vi "Enregis fichier local.vi"() -> ()   [LabVIEW 2022 SP3]
uses:
  Fichier local.ctl
  Enum/Enum f2l.ctl
  Fichier distant.ctl
  Variables globales/Variable glob generale.vi
panel:
  out "Fichier local":T1
  out "Ensemble données":string[](array[string])
  out "chemin local":path
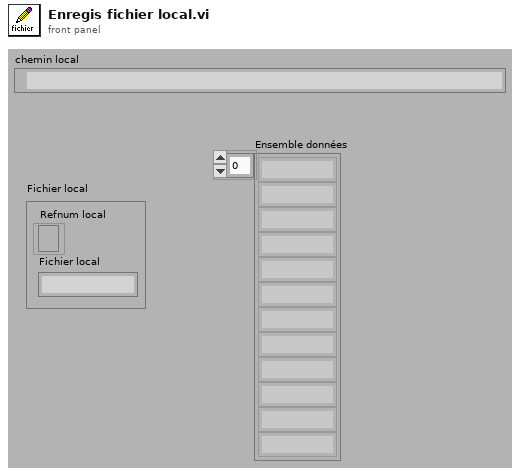
[diagram p1: front panel]
types:
  T1 = typedef "Fichier local.ctl" = cluster{"Refnum local":refnum<file>, "Fichier local":string}
  T2 = typedef "Enum f2l.ctl" = enum16{"Créer dossier local", "Créer fichier local", "Test date", "Test temps", "Données complètes", "Enregistrement"}
  T3 = enum16{"open", "replace", "create", "open or create", "replace or create", "replace or create with confirmation"}
  T4 = typedef "Fichier distant.ctl" = cluster{"refnum distant":refnum<file>, "Fichier distant":string}
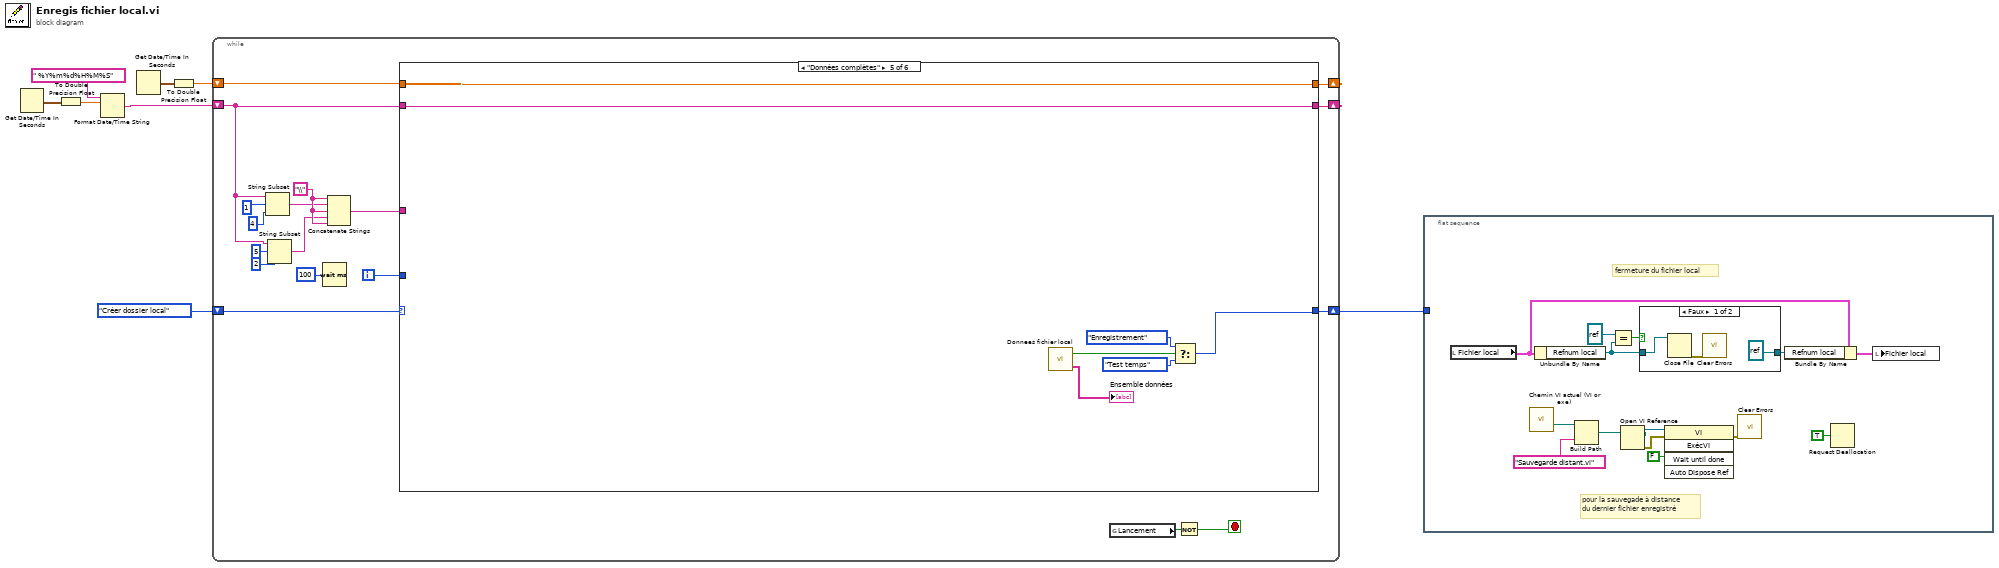
[diagram p0: block diagram]
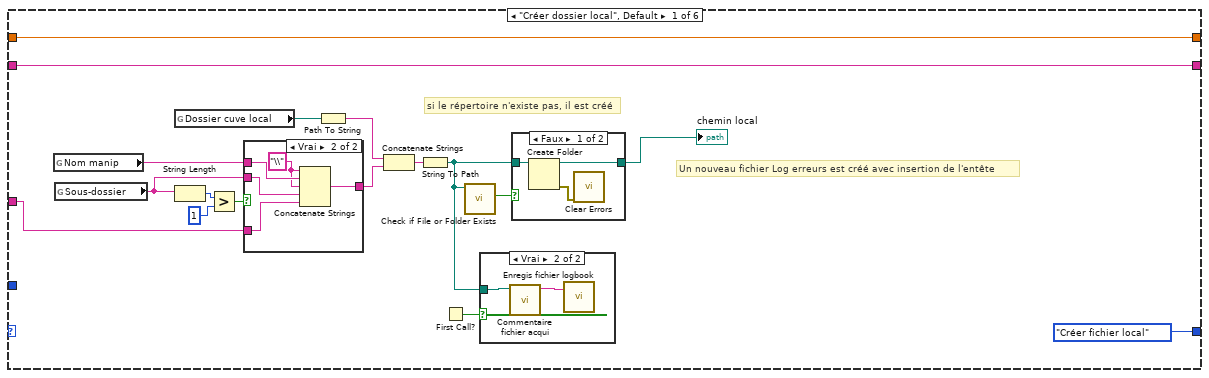
[diagram p3: hidden frame]
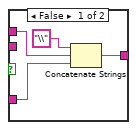
[diagram p5: hidden frame]
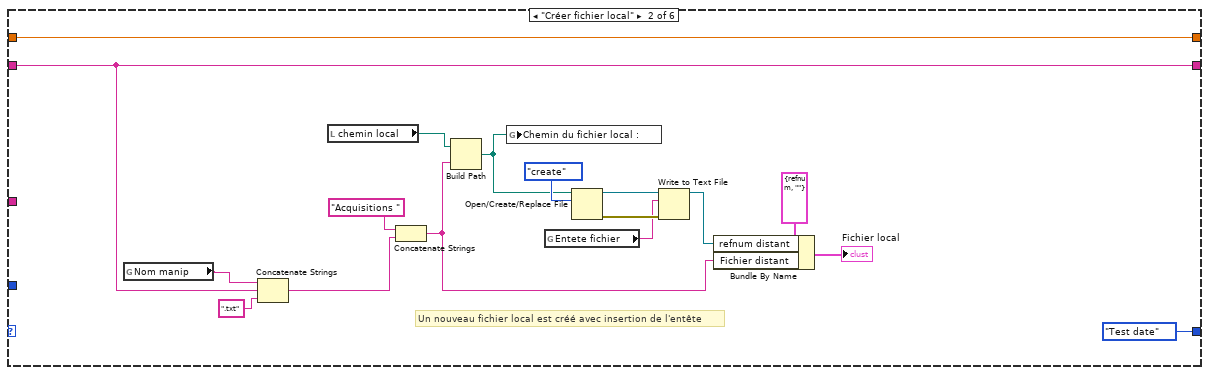
[diagram p7: hidden frame]
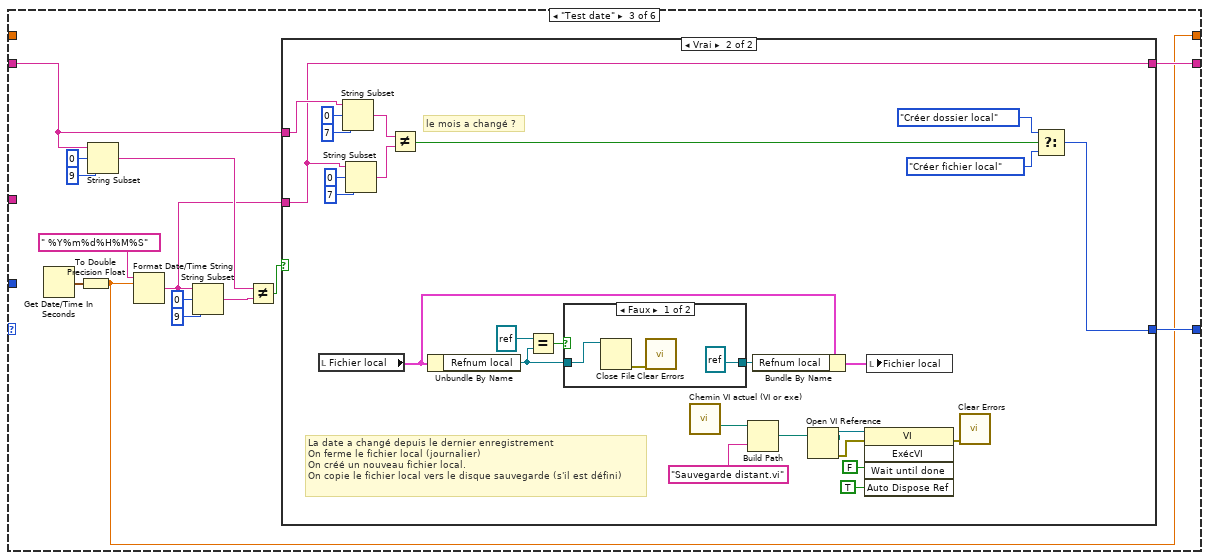
[diagram p8: hidden frame]
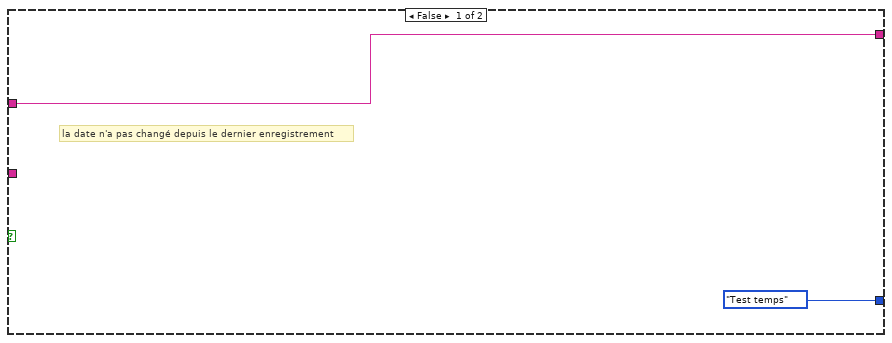
[diagram p9: hidden frame]
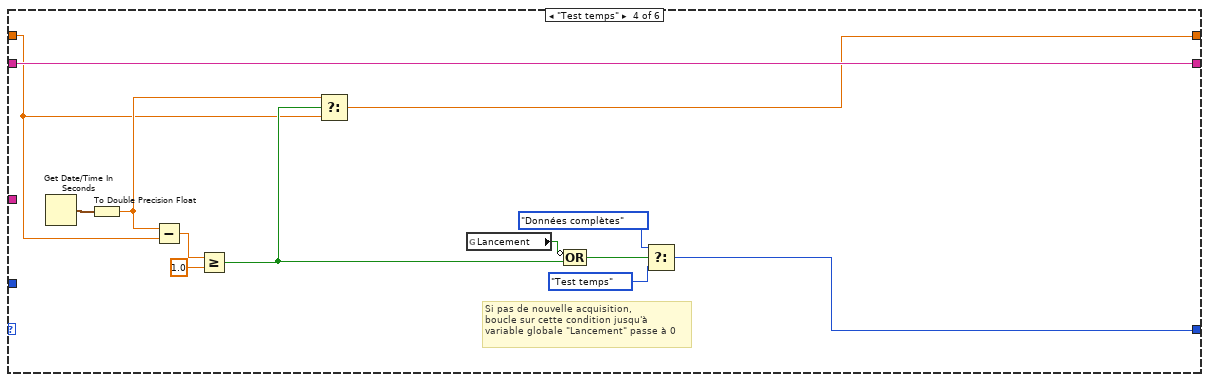
[diagram p11: hidden frame]
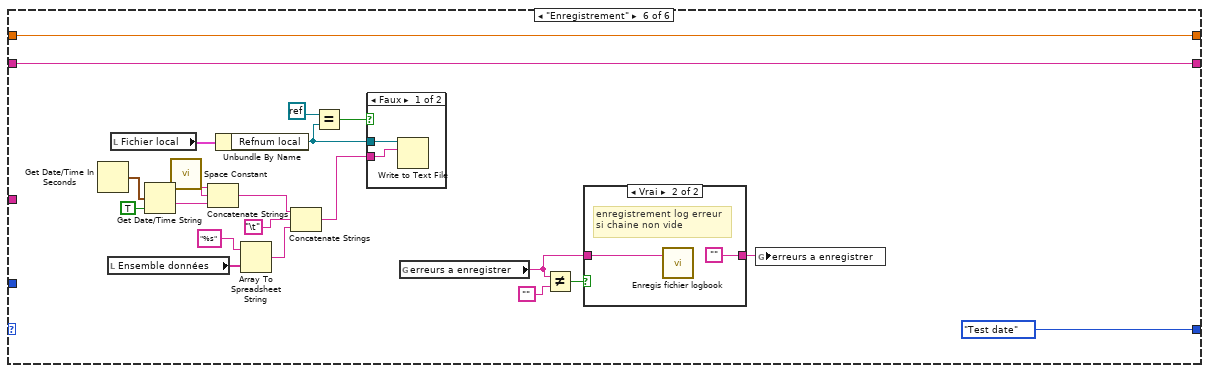
[diagram p12: hidden frame]
diagram:
  n1 = Get Date/Time In Seconds() -> (seconds since 1Jan1904=w7:timestamp)
  n2 = To Double Precision Float(number=w7) -> (double precision float=w5:dbl)
  n3 = Format Date/Time String(time format string (%c)=" %Y%m%d%H%M%S" ("chaîne de format de l'heure (%c)"), seconds (now)=w5) -> (date/time string=w4:string)  [unwired: 1 in]
  n4 = Get Date/Time In Seconds() -> (seconds since 1Jan1904=w3:timestamp)
  n5 = To Double Precision Float(number=w3) -> (double precision float=w2:dbl)
  n6 = while {
    shift-right: [w23] -> _
    shift-left: w4 -> [w13]
    shift-right: [w21] -> _
    shift-left: w2 -> [w22]
    shift-right: [w25] -> w1
    shift-left: Enum_f2l."Créer dossier local" ("Énum") -> [w26]
    i -> [w11]
    stop <- w9 stop-if-true
    w20 = "\\" ("chaîne")
    n7 = String Subset(string=w13, offset (0)=1, length (rest)=4 ("longueur (reste)")) -> (substring=w15:string)
    n8 = String Subset(string=w13, offset (0)=5, length (rest)=2 ("longueur (reste)")) -> (substring=w17:string)
    n9 = Wait (ms)(milliseconds to wait=u32 100 ("attente (ms)")) -> ()  [unwired: 1 out]
    n10 = Concatenate Strings(w20, w15, w20, w17, w20) -> (w12:string)
    n11 = case shown="\"Données complètes\"" w26 {
      tunnel: w12 -> [w34 _ _ _ _ _]
      tunnel: w13 -> [w31 w71 w83 w129 w139 w162]
      tunnel: [Enum_f2l."Créer fichier local" ("Énum") Enum_f2l."Test date" ("Énum") w86 w132 w141 Enum_f2l."Test date" ("Énum")] -> w25
      tunnel: [w31 w71 w85 w129 w139 w162] -> w23
      tunnel: w22 -> [w33 w74 _ w124 w140 w156]
      tunnel: [w33 w74 w84 w123 w140 w156] -> w21
      tunnel: w11 -> [_ _ _ _ _ _]
      frame "Créer dossier local", Default {
        # "Un nouveau fichier Log erreurs est créé avec insertion de l'entête"
        # "si le répertoire n'existe pas, il est créé"
        n12 = global read "Variable glob generale.vi" "Nom manip"() -> (w29:string)
        n13 = global read "Variable glob generale.vi" "Sous-dossier"() -> (w30:string)
        n14 = global read "Variable glob generale.vi" "Dossier cuve local"() -> (w39:path)
        n15 = String Length(string=w30) -> (length=w41:i32)
        n16 = Greater?(x=w41, y=1) -> (0:w40:bool)
        n17 = case shown="Vrai" w40 {
          tunnel: w29 -> [w48 w54]
          tunnel: w30 -> [_ w52]
          tunnel: w34 -> [w47 w51]
          tunnel: [w46 w50] -> w37
          frame False {
            n18 = Concatenate Strings("\\", w48, w47) -> (w46:string)
          }
          frame True {
            w53 = "\\"
            n19 = Concatenate Strings(w53, w54, w53, w52, w51) -> (w50:string)
          }
        }
        n20 = Path To String(path=w39) -> (string=w38:string)
        n21 = Concatenate Strings(w38, w37) -> (w36:string)
        n22 = String To Path(string=w36) -> (path=w27:path)
        n23 = First Call?() -> (First Call?: T/F=w28:bool)
        n24 = call <vilib>:"Check if File or Folder Exists.vi"("path"=w27) -> ("file or folder exists?"=w42:bool)  [unwired: 8 in, 2 out]
        n25 = case shown="Vrai" w28 {
          tunnel: w27 -> [_ w45]
          frame False {
          }
          frame True {
            n26 = call "Commentaire fichier acqui.vi"("Chemin"=w45) -> ("Chaîne"=w44:string)  [unwired: 10 in]
            n27 = call "Enregis fichier logbook.vi"("Chaîne"=w44) -> ()  [unwired: 2 in, 1 out]
          }
        }
        n28 = case shown="Faux" w42 {
          tunnel: w27 -> [w57 w58]
          tunnel: [w56 w58] -> w32
          frame False {
            n29 = Create Folder(path (use dialog)=w57) -> (created path=w56:path, error out=w55:errorcluster)  [unwired: 2 in, 1 out]
            n30 = call <vilib>:"Clear Errors.vi"("error in (no error)"=w55) -> ()  [unwired: 5 in, 2 out]
          }
          frame True {
          }
        }
        "chemin local" <- w32
      }
      frame "Créer fichier local" {
        # "Un nouveau fichier local est créé avec insertion de l'entête"
        n31 = global read "Variable glob generale.vi" "Nom manip"() -> (w73:string)
        n32 = Concatenate Strings(w73, w71, ".txt" ("chaîne")) -> (w61:string)
        n33 = local read "chemin local"() -> (w60:path)
        n34 = Concatenate Strings("Acquisitions ", w61) -> (w62:string)
        n35 = Build Path(base path=w60, name or relative path=w62) -> (appended path=w65:path)
        n36 = global write "Variable glob generale.vi" "Chemin du fichier local :"(w65) -> ()
        n37 = global read "Variable glob generale.vi" "Entete fichier"() -> (w59:string)
        n38 = Open/Create/Replace File(file path (use dialog)=w65, operation (0:open)=T3."create" ("opération (0 : open)")) -> (refnum out=w66:refnum<file>, error out=w67:errorcluster)  [unwired: 1 in, 4 out]
        n39 = Write to Text File(file (use dialog)=w66, text=w59, error in=w67) -> (refnum out=w70:refnum<file>)  [unwired: 1 in, 2 out]
        n40 = Bundle By Name(cluster=T4 {"refnum distant"=refnum, "Fichier distant"=""} ("Refnum File"), "refnum distant"=w70, "Fichier distant"=w62) -> (→"Fichier local":T4)
      }
      frame "Test date" {
        n41 = Get Date/Time In Seconds() -> (seconds since 1Jan1904=w88:timestamp)
        n42 = To Double Precision Float(number=w88) -> (double precision float=w84:dbl)
        n43 = String Subset(string=w83, offset (0)=0, length (rest)=9 ("longueur (reste)")) -> (substring=w78:string)
        n44 = Format Date/Time String(time format string (%c)=" %Y%m%d%H%M%S" ("chaîne de format de l'heure (%c)"), seconds (now)=w84) -> (date/time string=w76:string)  [unwired: 1 in]
        n45 = String Subset(string=w76, offset (0)=0, length (rest)=9 ("longueur (reste)")) -> (substring=w77:string)
        n46 = Not Equal?(x=w78, y=w77) -> (x != y?=w87:bool)
        n47 = case shown="Vrai" w87 {
          tunnel: [Enum_f2l."Test temps" ("Énum") w92] -> w86
          tunnel: w83 -> [w90 w99]
          tunnel: [w90 w98] -> w85
          tunnel: w76 -> [_ w98]
          frame False {
            # "la date n'a pas changé depuis le dernier enregistrement"
          }
          frame True {
            # "le mois a changé ?"
            # "La date a changé depuis le dernier enregistrement\nOn ferme le fichier local (journalier)\nOn créé un nouveau fichier local.\nOn copie le fichier local vers le disque sauvegarde (s'il est défini)"
            n48 = local read "Fichier local"() -> (w114:T1)
            n49 = String Subset(string=w99, offset (0)=0, length (rest)=7 ("longueur (reste)")) -> (substring=w97:string)
            n50 = String Subset(string=w98, offset (0)=0, length (rest)=7 ("longueur (reste)")) -> (substring=w96:string)
            n51 = Not Equal?(x=w97, y=w96) -> (x != y?=w95:bool)
            n52 = Unbundle By Name(w114) -> ("Refnum local"=w115:refnum<file>)
            n53 = Equal?(x=refnum<file> refnum, y=w115) -> (x = y?=w116:bool)
            n54 = case shown="Faux" w116 {
              tunnel: w115 -> [w120 w121]
              tunnel: [refnum<file> refnum ("x") w121] -> w113
              frame False {
                n55 = Close File(refnum=w120) -> (error out=w119:errorcluster)  [unwired: 1 in, 1 out]
                n56 = call <vilib>:"Clear Errors.vi"("error in (no error)"=w119) -> ()  [unwired: 5 in, 2 out]
              }
              frame True {
              }
            }
            n57 = call "Chemin VI actuel (VI or exe).vi"() -> ("VI or executable installation directory"=w111:path)  [unwired: 14 in, 1 out]
            n58 = Build Path(base path=w111, name or relative path="Sauvegarde distant.vi" ("nom ou chemin relatif")) -> (appended path=w106:path)
            n59 = Bundle By Name(cluster=w114, "Refnum local"=w113) -> (w112:T1)
            n60 = Open VI Reference(vi path=w106) -> (vi reference=w108:refnum<vi>, error out=w109:errorcluster)  [unwired: 5 in]
            n61 = invoke class="VI" method="ExécVI"(reference=w108, error in=w109, "Wait until done"=FALSE ("Attendre la fin"), "Auto Dispose Ref"=TRUE ("Supprimer la référence automatiquement")) -> (error out=w110:errorcluster)  [unwired: 1 in, 4 out]
            n62 = local write "Fichier local"(w112) -> ()
            n63 = call <vilib>:"Clear Errors.vi"("error in (no error)"=w110) -> ()  [unwired: 5 in, 2 out]
            n64 = Select(t=Enum_f2l."Créer dossier local" ("Énum"), s=w95, f=Enum_f2l."Créer fichier local" ("Énum")) -> (s? t:f=w92:T2)
          }
        }
      }
      frame "Test temps" {
        # "Si pas de nouvelle acquisition,\nboucle sur cette condition jusqu'à\nvariable globale \"Lancement\" passe à 0"
        n65 = Get Date/Time In Seconds() -> (seconds since 1Jan1904=w127:timestamp)
        n66 = To Double Precision Float(number=w127) -> (double precision float=w125:dbl)
        n67 = Subtract(x=w125, y=w124) -> (x-y=w128:dbl)
        n68 = Greater Or Equal?(x=w128, y=1.0) -> (x >= y?=w126:bool)
        n69 = Select(t=w125, s=w126, f=w124) -> (s? t:f=w123:dbl)
        n70 = global read "Variable glob generale.vi" "Lancement"() -> (w131:bool)
        n71 = Compound Arithmetic op=OR(invert w131, w126) -> (w130:bool)
        n72 = Select(t=Enum_f2l."Données complètes" ("Énum"), s=w130, f=Enum_f2l."Test temps" ("Énum")) -> (s? t:f=w132:T2)
      }
      frame "Données complètes" {
        n73 = call "Donnees fichier local.vi"() -> ("Données"=→"Ensemble données":string[], "données présentes"=w136:bool)  [unwired: 2 in]
        n74 = Select(t=Enum_f2l."Enregistrement" ("Énum"), s=w136, f=Enum_f2l."Test temps" ("Énum")) -> (s? t:f=w141:T2)
      }
      frame "Enregistrement" {
        n75 = Get Date/Time In Seconds() -> (seconds since 1Jan1904=w161:timestamp)
        n76 = local read "Ensemble données"() -> (w152:string[])
        n77 = local read "Fichier local"() -> (w155:T1)
        n78 = Get Date/Time String(seconds (now)=w161, want seconds? (F)=TRUE ("secondes ? (F)")) -> (date string=w159:string, time string=w158:string)  [unwired: 1 in]
        n79 = call <vilib>:"Space Constant.vi"() -> ("String"=w157:string)
        n80 = Concatenate Strings(w159, w157, w158) -> (w144:string)
        n81 = Unbundle By Name(w155) -> ("Refnum local"=w148:refnum<file>)
        n82 = Array To Spreadsheet String(array=w152, 3:"%s" ("chaîne de format")) -> (spreadsheet string=w150:string)  [unwired: 1 in]
        n83 = Concatenate Strings(w144, "\t", w150) -> (w147:string)
        n84 = Equal?(x=refnum<k0> refnum, y=w148) -> (x = y?=w153:bool)
        n85 = case shown="Faux" w153 {
          tunnel: w147 -> [w167 _]
          tunnel: w148 -> [w168 _]
          frame False {
            n86 = Write to Text File(file (use dialog)=w168, text=w167) -> ()  [unwired: 2 in, 3 out]
          }
          frame True {
          }
        }
        n87 = global read "Variable glob generale.vi" "erreurs a enregistrer"() -> (w143:string)
        n88 = Not Equal?(x=w143, y="") -> (x != y?=w145:bool)
        n89 = case shown="Vrai" w145 {
          tunnel: w143 -> [w164 w165]
          tunnel: [w164 ""] -> w142
          frame False {
          }
          frame True {
            # "enregistrement log erreur\nsi chaine non vide"
            n90 = call "Enregis fichier logbook.vi"("Chaîne"=w165) -> ()  [unwired: 2 in, 1 out]
          }
        }
        n91 = global write "Variable glob generale.vi" "erreurs a enregistrer"(w142) -> ()
      }
    }
    n92 = global read "Variable glob generale.vi" "Lancement"() -> (w10:bool)
    n93 = Not(x=w10) -> (.not. x?=w9:bool)
  }
  n94 = flat-sequence {
    tunnel: w1 -> [_]
    frame #0 {
      # "pour la sauvegade à distance\ndu dernier fichier enregistré"
      # "fermeture du fichier local"
      n95 = local read "Fichier local"() -> (w179:T1)
      n96 = call "Chemin VI actuel (VI or exe).vi"() -> ("VI or executable installation directory"=w169:path)  [unwired: 14 in, 1 out]
      n97 = Unbundle By Name(w179) -> ("Refnum local"=w178:refnum<file>)
      n98 = Build Path(base path=w169, name or relative path="Sauvegarde distant.vi" ("nom ou chemin relatif")) -> (appended path=w174:path)
      n99 = Equal?(x=refnum<file> refnum, y=w178) -> (x = y?=w177:bool)
      n100 = Open VI Reference(vi path=w174) -> (vi reference=w172:refnum<vi>, error out=w171:errorcluster)  [unwired: 5 in]
      n101 = case shown="Faux" w177 {
        tunnel: w178 -> [w185 w186]
        tunnel: [refnum<file> refnum ("x") w186] -> w180
        frame False {
          n102 = Close File(refnum=w185) -> (error out=w184:errorcluster)  [unwired: 1 in, 1 out]
          n103 = call <vilib>:"Clear Errors.vi"("error in (no error)"=w184) -> ()  [unwired: 5 in, 2 out]
        }
        frame True {
        }
      }
      n104 = invoke class="VI" method="ExécVI"(reference=w172, error in=w171, "Wait until done"=FALSE ("Attendre la fin")) -> (error out=w170:errorcluster)  [unwired: 2 in, 4 out]
      n105 = call <vilib>:"Clear Errors.vi"("error in (no error)"=w170) -> ()  [unwired: 5 in, 2 out]
      n106 = Bundle By Name(cluster=w179, "Refnum local"=w180) -> (w181:T1)
      n107 = Request Deallocation(TRUE ("flag")) -> ()
      n108 = local write "Fichier local"(w181) -> ()
    }
  }
